vi "Host Page In Panel.vi"(8 "error in (no error)":errorcluster, 9 "Node Ptr":T1 format="%.0x", 10 "VI Refnum in":refnum<vi>, 11 "SubPanel in":refnum<vi>) -> (0 "error out":errorcluster, 2 "VI Refnum out":refnum<vi>, 3 "SubPanel out":refnum<vi>)   [LabVIEW 2020, in "Engine Simulation Toolkit System Explorer.lvlib"]
uses:
  Engine Simulation Toolkit System Explorer.lvlib
  <vilib>/NI VeriStand/Custom Device API/Custom Device Item Ref.ctl
  <vilib>/NI VeriStand/Custom Device API/Custom Device API.lvlib
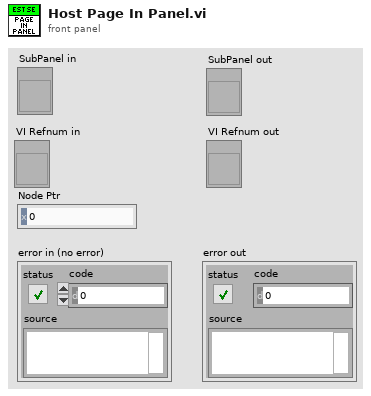
[diagram p1: front panel]
types:
  T1 = typedef "Custom Device API.lvlib/Custom Device Item Ref.ctl" = u64
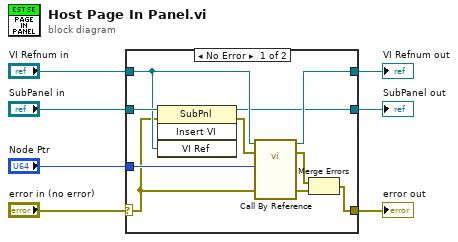
[diagram p0: block diagram]
diagram:
  n1 = case shown="No Error" "error in (no error)" {
    selector: "error in (no error)" -> [w11 w20]
    tunnel: [w10 w20] -> w7
    tunnel: "VI Refnum in" -> [w12 w18]
    tunnel: "SubPanel in" -> [w14 w19]
    tunnel: "Node Ptr" -> [w13 _]
    tunnel: [w9 w18] -> w2
    tunnel: [w8 w19] -> w1
    frame No Error {
      n2 = invoke on="Invoke Node" class="SubPnl" method="Insert VI"(reference=w14, error in=w11, "VI Ref"=w12) -> (reference out=w8:refnum<vi>, error out=w17:errorcluster)  [unwired: 1 in, 2 out]
      n3 = call-by-ref "?"(reference=w12, error in=w17, 8:"error in (no error)"=w11, "Node Ptr"=w13) -> (reference out=w9:refnum<vi>, error out=w16:errorcluster, 0:"error out"=w15:errorcluster)  [unwired: 9 in]
      n4 = Merge Errors(w16, w15) -> (w10:errorcluster)
    }
    frame Error {
    }
  }
  "error out" <- w7
  "VI Refnum out" <- w2
  "SubPanel out" <- w1
